vi "Send Configure Msg.vi"(8 "error in":errorcluster, 10 "analog generation":T1={"channel list"="", "output settings"={"output rate"=0.0, "range"=0.0, "terminal configuration"=enum."Pseudodifferential", "output impedance"=0.0, "common mode offset"=0.0, "pure tone mode"=FALSE}, "signal settings"={"signal type"=enum."Sine", "properties"=""}}, 11 "Qbus in":refnum<class "Qbus.lvclass">) -> (0 "error out":errorcluster, 3 "Qbus out":refnum<class "Qbus.lvclass">)   [LabVIEW 2021, in "AnalogGenerationProcess.lvlib"]
uses:
  AnalogGenerationProcess.lvlib
  <vilib>/addons/Qbus/Qbus.lvclass
  controls/analog generation settings.ctl
  controls/analog output settings.ctl
  controls/signal settings.ctl
  controls/signal type.ctl
  controls/AudioGenTypeDefs.lvlib
  controls/terminal configuration.ctl
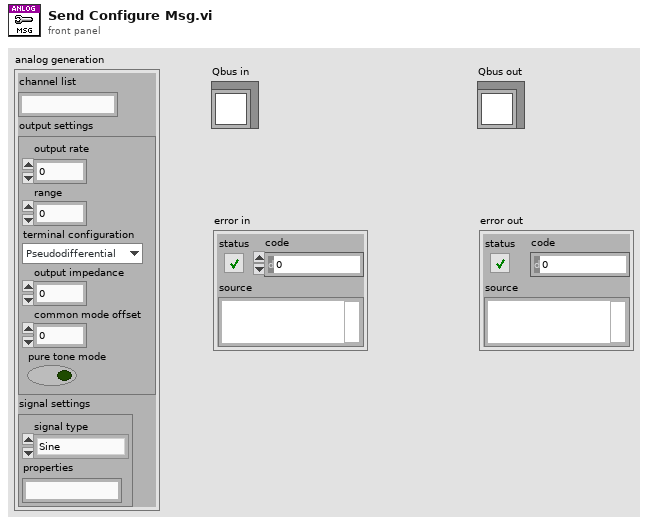
[diagram p1: front panel]
types:
  T1 = typedef "AudioGenTypeDefs.lvlib/analog generation settings.ctl" = cluster{"channel list":string, "output settings":T2, "signal settings":T4}
  T2 = typedef "AudioGenTypeDefs.lvlib/analog output settings.ctl" = cluster{"output rate":dbl, "range":dbl, "terminal configuration":T3, "output impedance":dbl, "common mode offset":dbl, "pure tone mode":bool}
  T3 = typedef "AudioGenTypeDefs.lvlib/terminal configuration.ctl" = enum32{"Default", "RSE", "Differential", "Pseudodifferential"}
  T4 = typedef "AudioGenTypeDefs.lvlib/signal settings.ctl" = cluster{"signal type":T5, "properties":string}
  T5 = typedef "AudioGenTypeDefs.lvlib/signal type.ctl" = enum16{"Sine", "Square", "Triangle", "White Noise", "Pink Noise", "Periodic Random Noise"}
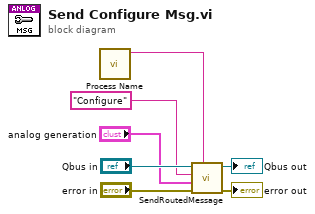
[diagram p0: block diagram]
diagram:
  n1 = call "Process Name.vi"() -> ("process name"=w2:string)  [unwired: 11 in]
  n2 = call <vilib>:"SendRoutedMessage.vi"("listener process"=w2, "error in (no error)"="error in", "message value"="analog generation", "message name"="Configure", "Qbus in"="Qbus in") -> ("error in (no error)"=→"error out":errorcluster, "Qbus out"=→"Qbus out":refnum<class "Qbus.lvclass">)  [unwired: 5 in]
